vi "Runtime Test.vi"() -> (0 "final error":errorcluster, 1 "correct execution settings":bool, 3 "Pass":bool)   [LabVIEW 2015, in "SystemLink File Module tests.lvlib"]
doc: "This VI shows an example for how to test the Runtime functionality of the module. This will need to be modified according to module functionality."
uses:
  SystemLink File Module tests.lvlib
  module/execution/SystemLink File runtime.lvclass
  <vilib>/NI/Tag Bus/dictionary/data dictionary.lvclass/data dictionary.ctl
  <vilib>/NI/Tag Bus/dictionary/lookup polymorphs/locate Boolean.vi
  <vilib>/NI/Tag Bus/table/data polymorphs/write one/write Boolean.vi
  <vilib>/NI/Tag Bus/dictionary/search/find data index.vi
  <vilib>/NI/Tag Bus/dictionary/search/search string list.vi
  <vilib>/Skyline/File/Filter/Create Filter (Name).vi
  <vilib>/NI/Tag Bus/dictionary/tag not found.vi
  module/configuration/SystemLink File configuration.lvclass
  <vilib>/NI/Tag Bus/dictionary/data dictionary.lvclass
  <vilib>/NI/Tag Bus/table/data table.lvlib
  <vilib>/Skyline/File/File/NI Skyline File.lvclass
  <vilib>/Skyline/File/Filter/NI Skyline File Filter.lvclass
panel:
  out "Names":string[](array[string])
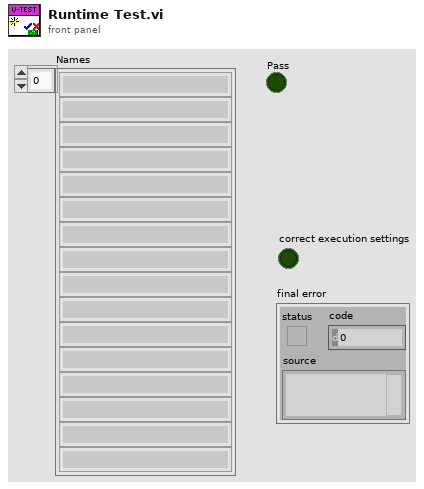
[diagram p1: front panel]
types:
  T1 = typedef "TBM channel.lvclass/data tables.ctl" = cluster{"input data":T2, "processing parameter":T2, "processing result":T2, "output data":T2}
  T2 = typedef "tag bus.lvlib/dictionary table pair.ctl" = cluster{"data dictionary":refnum<class "data dictionary.lvclass">, "data table":T3}
  T3 = typedef "tag bus.lvlib/data table.lvlib/data table.ctl" = cluster{"Double":dbl[], "Single":sgl[], "I64":i64[], "I32":i32[], "I16":i16[], "I8":i8[], "U64":u64[], "U32":u32[], "U16":u16[], "U8":u8[], "Boolean":bool[], "String":string[], "Array of Double":cluster{"DBL Array":dbl[]}[], "Array of Single":cluster{"SGL Array":sgl[]}[], "Array of I64":cluster{"I64 Array":i64[]}[], "Array of I32":cluster{"I32 Array":i32[]}[], "Array of I16":cluster{"I16 Array":i16[]}[], "Array of I8":cluster{"I8 Array":i8[]}[], "Array of U64":cluster{"U64 Array":u64[]}[], "Array of U32":cluster{"U32 Array":u32[]}[], "Array of U16":cluster{"U16 Array":u16[]}[], "Array of U8":cluster{"U8 Array":u8[]}[], "Array of Boolean":cluster{"Boolean Array":bool[]}[], "Array of String":cluster{"String Array":string[]}[]}
  T4 = typedef "TBM module execution interface.lvclass/execution settings.ctl" = cluster{"reads inputs":bool, "processes data":bool, "writes outputs":bool}
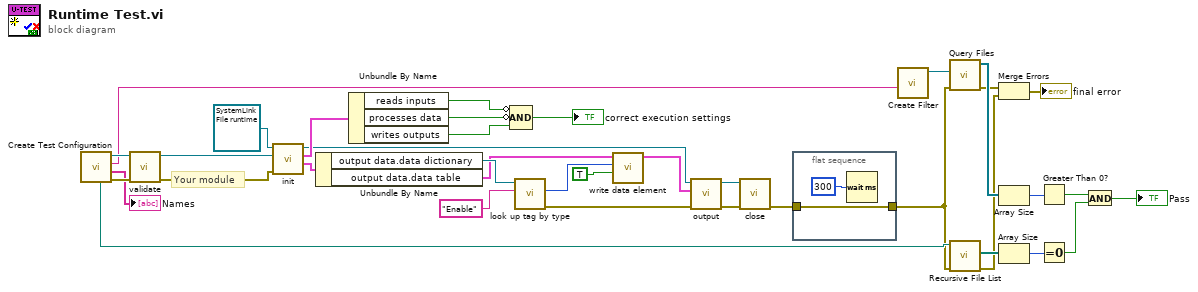
[diagram p0: block diagram]
diagram:
  # "Your module"
  n1 = call "Create Test Configuration.vi"() -> ("error out"=w27:errorcluster, "Names"=→"Names":string[], "File Name"=w14:string, "Module Configuration"=w28:refnum<class "SystemLink File configuration.lvclass">, "Folder Path"=w10:path)  [unwired: 5 in, 2 out]
  n2 = call-dynamic "validate.vi"("error in"=w27, "SystemLin Tag Module configuration in"=w28) -> ("error out"=w36:errorcluster, "SystemLin Tag Module configuration out"=w37:refnum<class "SystemLink File configuration.lvclass">)  [unwired: 8 in]
  n3 = call-dynamic "init.vi"("error in"=w36, "TBM module configuration in"=w37, "SystemLin Tag Module runtime in"=refnum<class "SystemLink File runtime.lvclass"> refnum ("tag bus configurable plugin module")) -> ("data allocations"=w29:T1, "execution settings"=w34:T4, "SystemLin Tag Module runtime out"=w25:refnum<class "SystemLink File runtime.lvclass">)  [unwired: 5 in, 1 out]
  n4 = Unbundle By Name(w29) -> ("output data.data dictionary"=w23:refnum<class "data dictionary.lvclass">, "output data.data table"=w19:T3)
  n5 = Unbundle By Name(w34) -> ("reads inputs"=w31:bool, "processes data"=w33:bool, "writes outputs"=w32:bool)
  n6 = Compound Arithmetic op=AND(invert w31, invert w33, w32) -> (→"correct execution settings":bool)
  n7 = call-poly <vilib>:"look up tag by type.vi"("name"="Enable" ("channel name"), "data dictionary in"=w23) -> ("error out"=w17:errorcluster, "index"=w21:i32)  [unwired: 7 in, 1 out]
  n8 = call-poly <vilib>:"write data element.vi"("value"=TRUE, "index"=w21, "data table in"=w19) -> ("data table out"=w18:T3)  [unwired: 8 in]
  n9 = call-dynamic "output.vi"("error in"=w17, "data table in"=w18, "SystemLin Tag Module runtime in"=w25) -> ("error out"=w16:errorcluster, "SystemLin Tag Module runtime out"=w24:refnum<class "SystemLink File runtime.lvclass">)  [unwired: 6 in, 1 out]
  n10 = call-dynamic "close.vi"("error in"=w16, "SystemLin Tag Module runtime in"=w24) -> ("error out"=w11:errorcluster)  [unwired: 9 in]
  n11 = flat-sequence {
    tunnel: [w38] -> w4
    tunnel: w11 -> [w38]
    frame #0 {
      n12 = Wait (ms)(milliseconds to wait=u32 300) -> ()  [unwired: 1 out]
    }
  }
  n13 = call-poly <vilib>:"Create Filter.vi"("value"=w14) -> ("filter out"=w15:refnum<class "NI Skyline File Filter.lvclass">)  [unwired: 9 in, 1 out]
  n14 = call <vilib>:"Query Files.vi"("error in (no error)"=w4, "filter"=w15) -> ("error out"=w3:errorcluster, "available files"=w13:refnum<class "NI Skyline File.lvclass">[])  [unwired: 7 in, 1 out]
  n15 = call <vilib>:"Recursive File List.vi"("error in (no error)"=w4, "Folder Path"=w10) -> ("error out"=w2:errorcluster, "All Files in Dir"=w9:path[])  [unwired: 5 in, 3 out]
  n16 = Merge Errors(w3, w2) -> (→"final error":errorcluster)
  n17 = Array Size(array=w13) -> (size(s)=w12:i32)
  n18 = Array Size(array=w9) -> (size(s)=w8:i32)
  n19 = Greater Than 0?(x=w12) -> (x > 0?=w6:bool)
  n20 = Equal To 0?(x=w8) -> (x = 0?=w7:bool)
  n21 = And(x=w6, y=w7) -> (x .and. y?=→"Pass":bool)
